vi "Chrome.vi"() -> ()   [LabVIEW 2026]
doc: "Uses a Web Browser to display web content."
uses:
  <vilib>/MediaMongrels Ltd/WebSockets/WebSockets/WebSocket/WebSocket.lvclass/WebSocket.ctl
  <vilib>/MediaMongrels Ltd/WebSockets/WebSockets/WebSocket Server/WebSocket Server.lvclass/WebSocket Server.ctl
  <vilib>/MediaMongrels Ltd/WebSockets/WebSockets/WebSocket/Read Return Headers.vi
  <vilib>/MediaMongrels Ltd/WebSockets/WebSockets/WebSocket Server/Read Request URI.vi
  <vilib>/MediaMongrels Ltd/WebSockets/WebSockets/WebSocket Server/WebSocket Server.lvclass
  C:/Program Files/National Instruments/LabVIEW 2026/vi.lib/MediaMongrels Ltd/WebSockets/WebSockets/WebSocket/WebSocket.lvclass
  <vilib>/MediaMongrels Ltd/WebSockets/Sockets/VISA TCP Listener/VISA TCP Listener.lvclass
panel:
  in  "Websocket Port":u16=8081
  in  "To Web Page":u16
  out "Request URI":string
  out "HTTP Headers":variant
  out "From Web Page":u16
  in  "Stop":bool
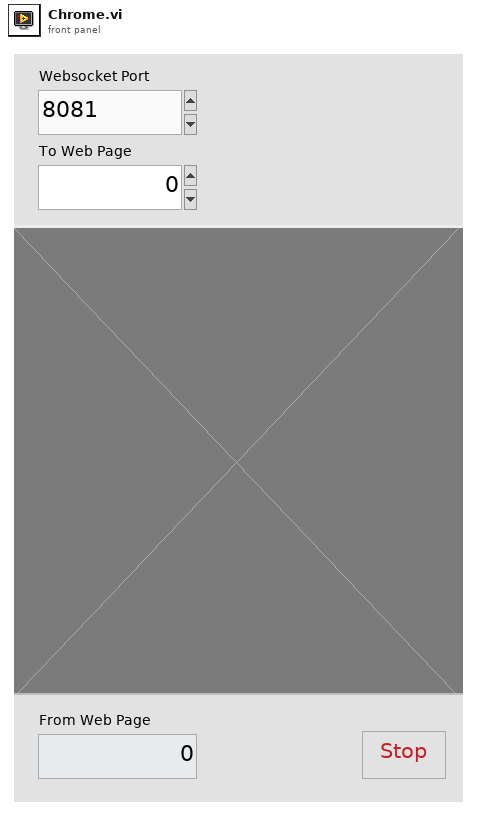
[diagram p1: front panel]
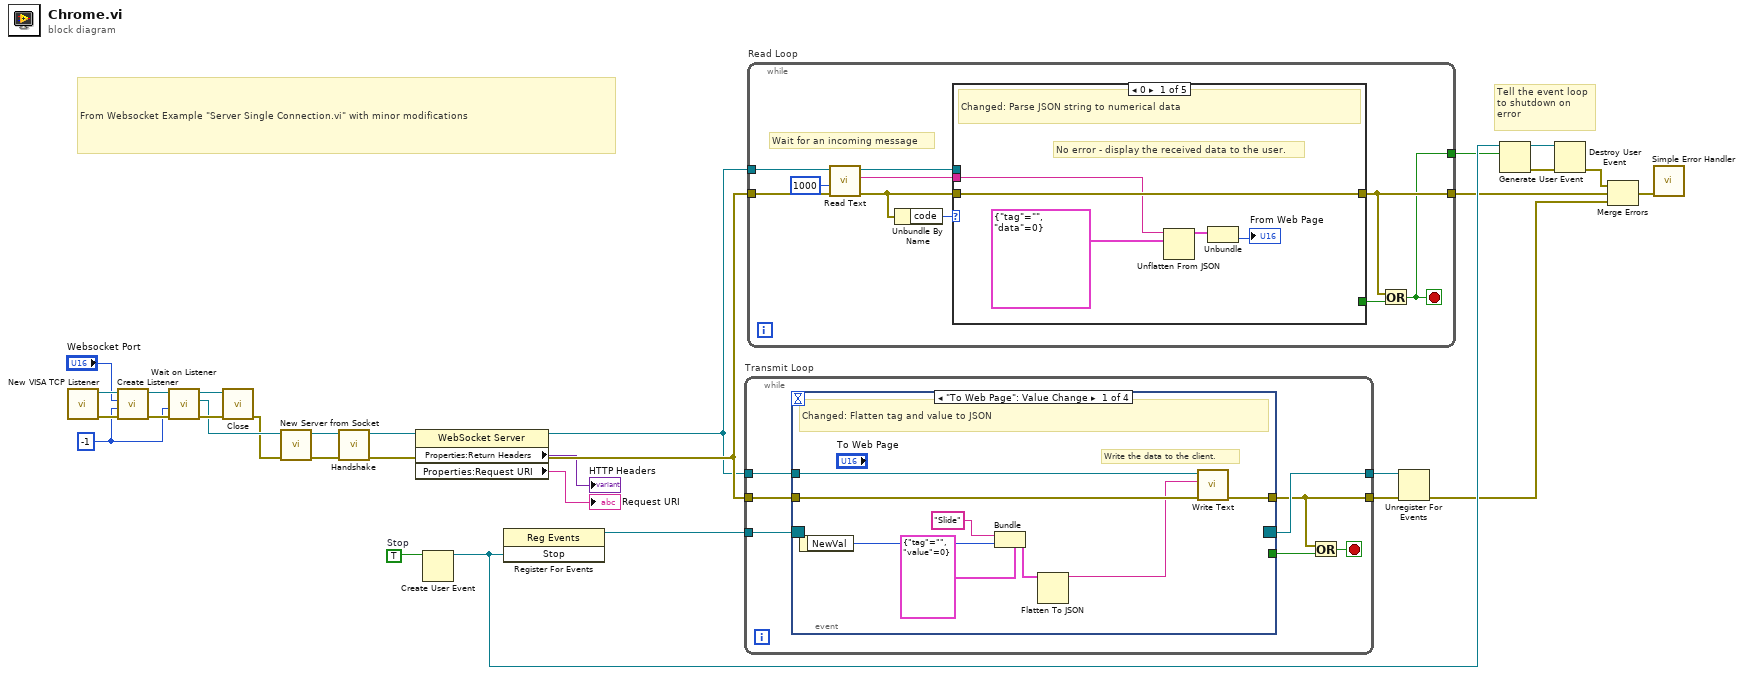
[diagram p0: block diagram]
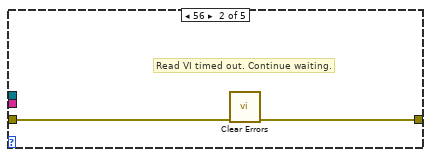
[diagram p2: hidden frame]
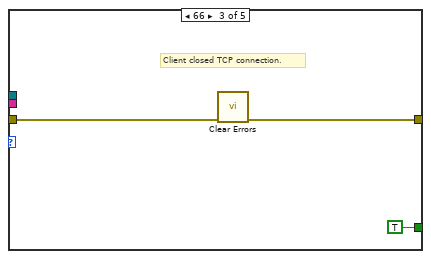
[diagram p3: hidden frame]
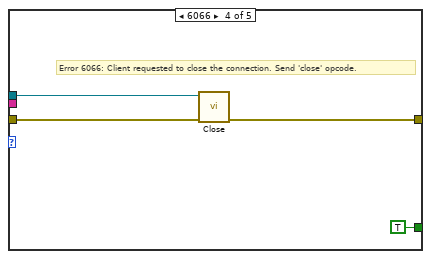
[diagram p4: hidden frame]
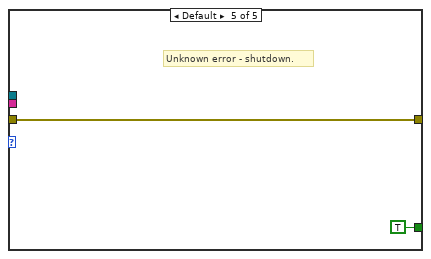
[diagram p5: hidden frame]
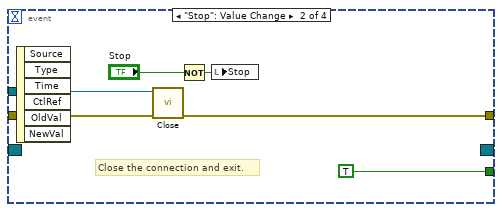
[diagram p6: hidden frame]
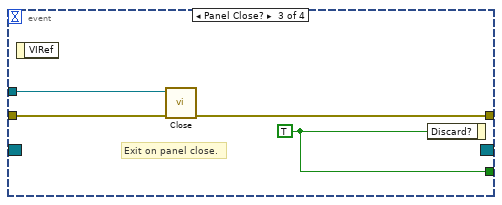
[diagram p7: hidden frame]
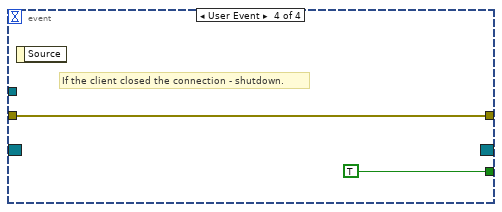
[diagram p8: hidden frame]
diagram:
  w20 = TRUE  # Stop
  w23 = -1 ("timeout ms (25000)")
  # "From Websocket Example \"Server Single Connection.vi\" with minor modifications"
  # "Tell the event loop to shutdown on error"
  n1 = call <vilib>:"New VISA TCP Listener.vi"() -> ("error out"=w29:errorcluster, "VISA TCP Listener out"=w30:refnum<class "VISA TCP Listener.lvclass">)  [unwired: 10 in]
  n2 = call-dynamic "Create Listener.vi"("error in (no error)"=w29, "timeout ms (5000)"=w23, "Port"="Websocket Port", "VISA TCP Listener in"=w30) -> ("error out"=w27:errorcluster, "VISA TCP Listener out"=w25:refnum<class "VISA TCP Listener.lvclass">)  [unwired: 6 in]
  n3 = call-dynamic "Wait on Listener.vi"("error in (no error)"=w27, "timeout ms (5000)"=w23, "VISA TCP Listener in"=w25) -> ("error out"=w28:errorcluster, "Socket out"=w22:refnum<class "Socket.lvclass">, "VISA TCP Listener out"=w26:refnum<class "VISA TCP Listener.lvclass">)  [unwired: 6 in]
  n4 = call-dynamic "Close.vi"("error in (no error)"=w28, "VISA TCP Listener in"=w26) -> ("error out"=w7:errorcluster)  [unwired: 9 in]
  n5 = call <vilib>:"New Server from Socket.vi"("error in (no error)"=w7, "Socket"=w22) -> ("error out"=w3:errorcluster, "WebSocket Server out"=w5:refnum<class "WebSocket Server.lvclass">)  [unwired: 8 in]
  n6 = call-dynamic "Handshake.vi"("error in (no error)"=w3, "WebSocket Connection in"=w5) -> ("error out"=w2:errorcluster, "WebSocket Connection out"=w4:refnum<class "WebSocket Server.lvclass">)  [unwired: 8 in]
  n7 = property class="WebSocket Server"(reference=w4, error in=w2) -> (reference out=w8:refnum<class "WebSocket Server.lvclass">, error out=w9:errorcluster, "Properties:Return Headers"=→"HTTP Headers":variant, "Properties:Request URI"=→"Request URI":string)
  n8 = Create User Event(user event datatype=w20) -> (user event=w18:refnum<user-event>)  [unwired: 1 in, 1 out]
  n9 = register-events(w18) -> (reference out=w21:refnum<event-registration>)  [unwired: 2 in, 1 out]
  n10 = while "Transmit Loop" {
    tunnel: w8 -> [w37]
    tunnel: w21 -> [w36]
    tunnel: [w35] -> w19
    tunnel: [w31] -> w12
    tunnel: w9 -> [w34]
    stop <- w32 stop-if-true
    n11 = event shown="[0] \"To Web Page\": Value Change" {
      selector: w36 -> [_ _ _ _]
      dyn-events: [_ _ _ _] -> w35
      timeout: _ -> [_ _ _ _]
      tunnel: w37 -> [w45 w50 w55 _]
      tunnel: [_ TRUE w54 TRUE] -> w33
      tunnel: [w43 w49 w53 w56] -> w31
      tunnel: w34 -> [w44 w48 w52 w56]
      event "To Web Page": Value Change {
        # "Write the data to the client."
        # "Changed: Flatten tag and value to JSON"
        n12 = event-data() -> ("NewVal"=w39:u16)  [unwired: 1 in]
        n13 = Bundle(cluster=cluster{"tag":string, "value":u16} {"tag"="", "value"=0}, "tag"="Slide", "value"=w39) -> (w42:cluster{"tag":string, "value":u16})
        n14 = Flatten To JSON(anything=w42) -> (JSON string=w38:string)  [unwired: 2 in, 1 out]
        n15 = call-dynamic "Write Text.vi"("error in (no error)"=w44, "String Data"=w38, "WebSocket in"=w45) -> ("error out"=w43:errorcluster)  [unwired: 7 in, 1 out]
      }
      event "Stop": Value Change {
        # "Close the connection and exit."
        n16 = event-data() -> ()  [unwired: 1 in, 6 out]
        n17 = call-dynamic "Close.vi"("error in (no error)"=w48, "WebSocket in"=w50) -> ("error out"=w49:errorcluster)  [unwired: 9 in]
        n18 = Not(x="Stop") -> (.not. x?=w47:bool)
        n19 = local write "Stop"(w47) -> ()
      }
      event Panel Close? {
        w54 = TRUE ("Discard?")
        # "Exit on panel close."
        n20 = event-data() -> ()  [unwired: 1 in, 1 out]
        n21 = call-dynamic "Close.vi"("error in (no error)"=w52, "WebSocket in"=w55) -> ("error out"=w53:errorcluster)  [unwired: 9 in]
        n22 = event-data("Discard?"=w54) -> ()  [unwired: 1 in, 1 out]
      }
      event User Event {
        # "If the client closed the connection - shutdown."
        n23 = event-data() -> ()  [unwired: 1 in, 1 out]
      }
    }
    n24 = Or(x=w31, y=w33) -> (x .or. y?=w32:bool)
  }
  n25 = while "Read Loop" {
    tunnel: w8 -> [w67]
    tunnel: [w58] -> w17
    tunnel: [w60] -> w11
    tunnel: w9 -> [w61]
    stop <- w58 stop-if-true
    # "Wait for an incoming message"
    n26 = call-dynamic "Read Text.vi"("error in (no error)"=w61, "timeout ms (5000)"=1000 ("timeout ms (25000)"), "WebSocket in"=w67) -> ("error out"=w62:errorcluster, "Data"=w64:string, "WebSocket out"=w63:refnum<class "WebSocket Server.lvclass">)  [unwired: 6 in]
    n27 = Unbundle By Name(w62) -> ("code"=w65:i32)
    n28 = case shown="0" w65 {
      tunnel: w64 -> [w71 _ _ _ _]
      tunnel: [_ _ TRUE TRUE TRUE] -> w59
      tunnel: w63 -> [_ _ _ w81 _]
      tunnel: w62 -> [w72 w74 w76 w79 w82]
      tunnel: [w72 w73 w75 w78 w82] -> w60
      frame 0 {
        # "No error - display the received data to the user."
        # "Changed: Parse JSON string to numerical data"
        n29 = Unflatten From JSON(JSON string=w71, type and defaults=cluster{"tag":string, "data":u16} {"tag"="", "data"=0}) -> (value=w69:cluster{"tag":string, "data":u16})  [unwired: 5 in, 1 out]
        n30 = Unbundle(w69) -> ("data"=→"From Web Page":u16)  [unwired: 1 out]
      }
      frame 56 {
        # "Read VI timed out. Continue waiting."
        n31 = call <vilib>:"Clear Errors.vi"("error in (no error)"=w74) -> ("error out"=w73:errorcluster)  [unwired: 5 in, 1 out]
      }
      frame 66 {
        # "Client closed TCP connection."
        n32 = call <vilib>:"Clear Errors.vi"("error in (no error)"=w76) -> ("error out"=w75:errorcluster)  [unwired: 5 in, 1 out]
      }
      frame 6066 {
        # "Error 6066: Client requested to close the connection. Send 'close' opcode."
        n33 = call-dynamic "Close.vi"("error in (no error)"=w79, "WebSocket in"=w81) -> ("error out"=w78:errorcluster)  [unwired: 9 in]
      }
      frame Default {
        # "Unknown error - shutdown."
      }
    }
    n34 = Or(x=w60, y=w59) -> (x .or. y?=w58:bool)
  }
  n35 = Unregister For Events(event registration refnum=w19, error in=w12) -> (error out=w10:errorcluster)
  n36 = Generate User Event(user event=w18, event data cluster=w17) -> (user event out=w16:refnum<user-event>, error out=w15:errorcluster)  [unwired: 2 in]
  n37 = Destroy User Event(user event=w16, error in=w15) -> (error out=w14:errorcluster)
  n38 = Merge Errors(w14, w11, w10) -> (w13:errorcluster)
  n39 = call <vilib>:"Simple Error Handler.vi"("error in (no error)"=w13) -> ()  [unwired: 4 in, 5 out]
